vi "ClassAttributes_GetClassAttributes_4x4x4.vi"(8 "error in":errorcluster, 10 "OnlyGetDvrReference(False)":bool, 11 "reference in":refnum<class>) -> (0 "error out":errorcluster, 1 "Class attribute Reference":refnum<data-value>, 2 "Class attribute":T1, 3 "reference out":refnum<class>)   [LabVIEW 2020]
doc: "Returns the class attributes of this class or a sub class. If reference is wired, the class attributes of the class (or sub class) will be returned else the class attributes will default to this class.\n\nIf the data is currently locked for modification, 'Attributes locked?' will return TRUE. If reference is wired, the class attributes of this class (or sub class) will be returned else the class attributes of this class."
uses:
  ClassAttributes_ClassAttributes.ctl
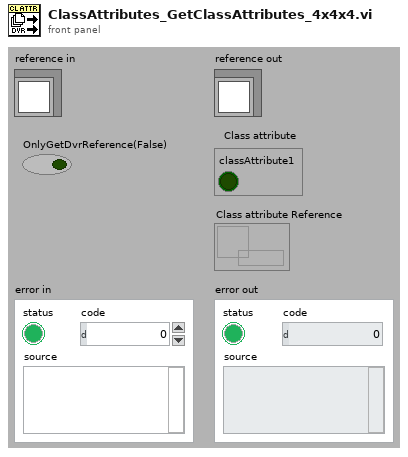
[diagram p1: front panel]
types:
  T1 = typedef "ClassAttributes_ClassAttributes.ctl" = cluster{"classAttribute1":bool}
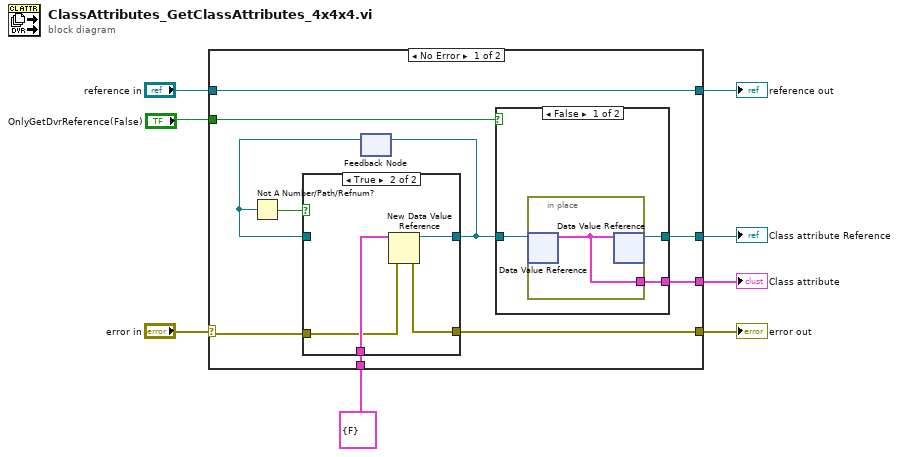
[diagram p0: block diagram]
diagram:
  n1 = case shown="No Error" "error in" {
    selector: "error in" -> [w16 w30]
    tunnel: [w18 w31] -> w8
    tunnel: [w15 w30] -> w7
    tunnel: "reference in" -> [w18 w31]
    tunnel: T1 {"classAttribute1"=FALSE} ("Class attributes") -> [w17 _]
    tunnel: [w14 _] -> w3
    tunnel: [w13 _] -> w2
    tunnel: "OnlyGetDvrReference(False)" -> [w9 _]
    frame No Error {
      n2 = feedback #1() -> (w10:refnum<data-value>)  [unwired: 1 in]
      n3 = Not A Number/Path/Refnum?(number/path/refnum=w10) -> (NaN/Path/Refnum?=w11:bool)
      n4 = case shown="True" w11 {
        tunnel: w17 -> [_ w29]
        tunnel: w16 -> [w24 w27]
        tunnel: [w24 w26] -> w15
        tunnel: [w25 w28] -> w12
        tunnel: w10 -> [w25 _]
        frame False {
        }
        frame True {
          n5 = New Data Value Reference(data value=w29, error in=w27) -> (data value reference=w28:refnum<data-value>, error out=w26:errorcluster)
        }
      }
      n6 = feedback-in #1(w12) -> ()
      n7 = case shown="False" w9 {
        tunnel: [w21 w23] -> w14
        tunnel: [w20 _] -> w13
        tunnel: w12 -> [w19 w23]
        frame False {
          n8 = in-place {
            in-place-border: [w22] -> w20
            n9 = in-place-dvr #2(w19) -> (w22:T1)  [unwired: 1 out]
            n10 = in-place-dvr #2(w22) -> (w21:refnum<data-value>)  [unwired: 1 out]
          }
        }
        frame True {
        }
      }
    }
    frame Error {
    }
  }
  "error out" <- w7
  "reference out" <- w8
  "Class attribute" <- w2
  "Class attribute Reference" <- w3
